vi "Scale Channel (Array).vi"(9 "Data":dbl[](array[numeric]), 10 "Scaling Params":dbl[](array[numeric]), 11 "Scaling Type":T1) -> (1 "Scaled Data":dbl[](array[numeric]))   [LabVIEW 2020, in "VolatusData.lvlib" / "Scaling.lvclass"]
uses:
  Scaling.lvclass
  VolatusConfig/Scale Type.ctl
  Scaling.lvclass/Scaling.ctl
  VolatusConfig/VolatusConfig.lvlib
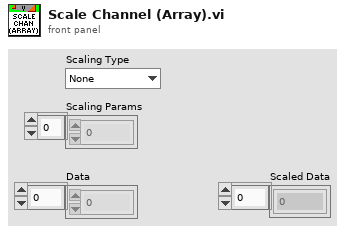
[diagram p1: front panel]
types:
  T1 = typedef "VolatusConfig.lvlib/Scale Type.ctl" = enum16{"None", "Sensor", "Polynomial", "Threshold", "Invert Bool", "Exponential"}
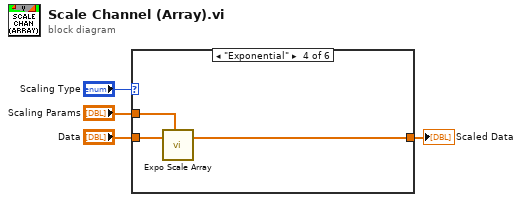
[diagram p0: block diagram]
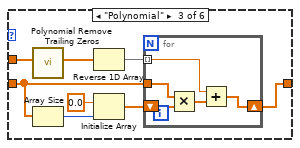
[diagram p4: hidden frame]
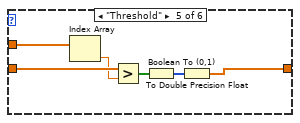
[diagram p5: hidden frame]
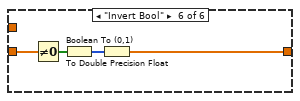
[diagram p6: hidden frame]
diagram:
  n1 = case shown="\"Exponential\"" "Scaling Type" {
    tunnel: "Scaling Params" -> [_ _ w13 w21 w28 _]
    tunnel: "Data" -> [w5 w6 w9 w22 w27 w32]
    tunnel: [w5 w6 w7 w20 w23 w29] -> w1
    frame "None" {
    }
    frame "Sensor" {
      # "#ERROR?\nSensor should be converted to another type. At least keep raw value passed through to be displayed and logged."
    }
    frame "Polynomial" {
      n2 = call "Polynomial Remove Trailing Zeros.vi"("Coefficients"=w13) -> ("Used Coefficients"=w14:dbl[])  [unwired: 10 in]
      n3 = Array Size(array=w9) -> (size(s)=w12:i32)
      n4 = Reverse 1D Array(array=w14) -> (reversed array=w8:dbl[])
      n5 = Initialize Array(0.0 ("element"), w12) -> (w10:dbl[])
      n6 = for {
        shift-right: [w15] -> w7
        shift-left: w10 -> [w19]
        tunnel: w9 -> [w18]
        tunnel: w8 -> [w16] mode=indexing
        n7 = Multiply(x=w18, y=w19) -> (x*y=w17:dbl[])
        n8 = Add(x=w16, y=w17) -> (x+y=w15:dbl[])
      }
    }
    frame "Exponential" {
      n9 = call "Expo Scale Array.vi"("Data"=w22, "Params"=w21) -> ("Scaled Data"=w20:dbl[])  [unwired: 5 in]
    }
    frame "Threshold" {
      n10 = Index Array(array=w28) -> (element=w26:dbl)  [unwired: 1 in]
      n11 = Greater?(x=w27, y=w26) -> (0:w25:bool[])
      n12 = Boolean To (0,1)(Boolean=w25) -> (0, 1=w24:i16[])
      n13 = To Double Precision Float(number=w24) -> (double precision float=w23:dbl[])
    }
    frame "Invert Bool" {
      n14 = Not Equal To 0?(x=w32) -> (x != 0?=w31:bool[])
      n15 = Boolean To (0,1)(Boolean=w31) -> (0, 1=w30:i16[])
      n16 = To Double Precision Float(number=w30) -> (double precision float=w29:dbl[])
    }
  }
  "Scaled Data" <- w1
